vi "Construct Listbox Item Names Binding.vi"(9 "Set to top upon write? (F)":T1, 10 "LstBox Refnum":refnum<vi>) -> (0 "error out":errorcluster, 3 "ListboxItemNamesBinding":refnum<class "ListboxItemNamesBinding.lvclass">)   [LabVIEW 2018, in "MVA Framework.lvlib" / "ListboxItemNamesBinding.lvclass"]
doc: "构造列表框项名绑定"
uses:
  ListboxItemNamesBinding.lvclass
  <vilib>/ErrorRing/Error Ring.xnode
  <vilib>/Utility/error.llb/Error Cluster From Error Code.vi
  Listbox Binding Options.ctl
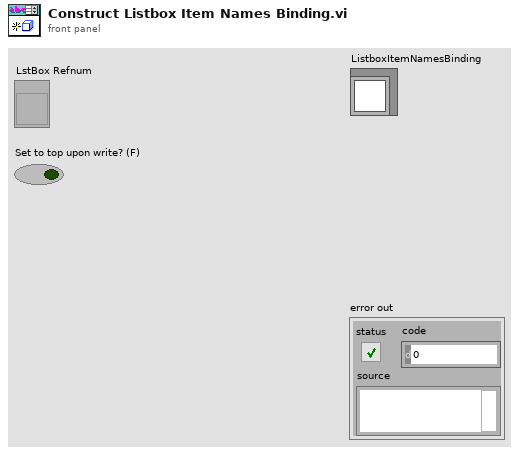
[diagram p1: front panel]
types:
  T1 = typedef "MVA Framework.lvlib/ListboxItemNamesBinding.lvclass/Listbox Binding Options.ctl" = bool
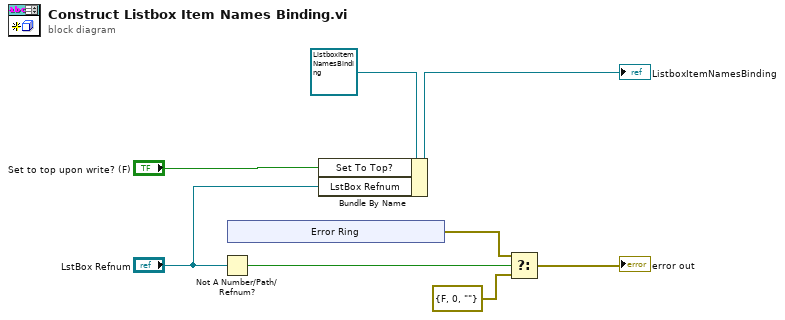
[diagram p0: block diagram]
diagram:
  n1 = Not A Number/Path/Refnum?(number/path/refnum="LstBox Refnum") -> (NaN/Path/Refnum?=w4:bool)
  n2 = xnode "Error Ring"() -> ("错误输出"=w1:errorcluster)
  n3 = Bundle By Name(cluster=refnum<class "ListboxItemNamesBinding.lvclass"> refnum ("ListboxItemNamesBinding"), "Set To Top?"="Set to top upon write? (F)", "LstBox Refnum"="LstBox Refnum") -> (→"ListboxItemNamesBinding":refnum<class "ListboxItemNamesBinding.lvclass">)
  n4 = Select(t=w1, s=w4, f=errorcluster {"status"=FALSE, "code"=0, "source"=""} ("error constant")) -> (s? t:f=→"error out":errorcluster)
